vi "FGV Sine User Event.vi"() -> (0 "error out":errorcluster, 3 "User Event out":refnum<user-event>)   [LabVIEW 2026]
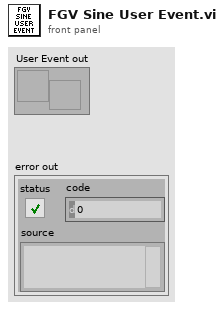
[diagram p1: front panel]
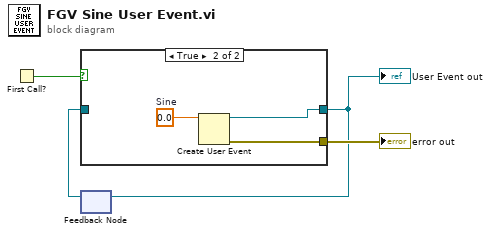
[diagram p0: block diagram]
diagram:
  n1 = First Call?() -> (First Call?: T/F=w1:bool)
  n2 = feedback #1() -> (w2:refnum<user-event>)  [unwired: 1 in]
  n3 = case shown="True" w1 {
    tunnel: [w5 w8] -> w3
    tunnel: [_ w6] -> w4
    tunnel: w2 -> [w5 _]
    frame False {
    }
    frame True {
      w7 = 0.0  # Sine
      n4 = Create User Event(user event datatype=w7) -> (user event=w8:refnum<user-event>, error out=w6:errorcluster)  [unwired: 1 in]
    }
  }
  "User Event out" <- w3
  "error out" <- w4
  n5 = feedback-in #1(w3) -> ()
